vi "libssh2_knownhost_readfile.vi"(8 "error in (no error)":errorcluster, 9 "type (OpenSSH)":T1, 10 "filename":path, 11 "host key database":T2) -> (0 "error out":errorcluster, 2 "hosts added":i32)   [LabVIEW 2017, in "libssh2.lvlib"]
doc: "Read host keys from a file and add them to a host key database."
uses:
  libssh2.lvlib
  Host Key Database Refnum.ctl
  Host Key File Type.ctl
  Not A Host Key Database.vi
  <vilib>/Utility/error.llb/Error Cluster From Error Code.vi
  Global Settings.vi
  Read Host Key Database Refnum.vi
  <vilib>/Utility/semaphor.llb/Acquire Semaphore.vi
  <vilib>/Utility/semaphor.llb/Release Semaphore.vi
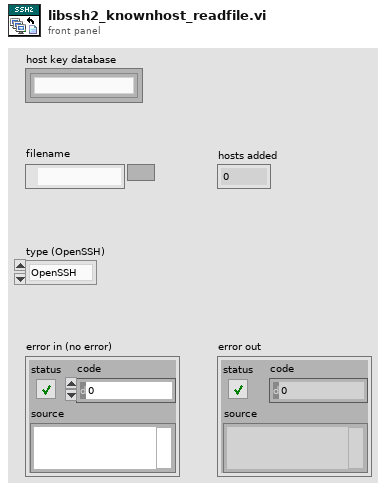
[diagram p1: front panel]
types:
  T1 = typedef "libssh2.lvlib/Host Key File Type.ctl" = enum16{"OpenSSH"}
  T2 = typedef "libssh2.lvlib/Host Key Database Refnum.ctl" = refnum<k1>
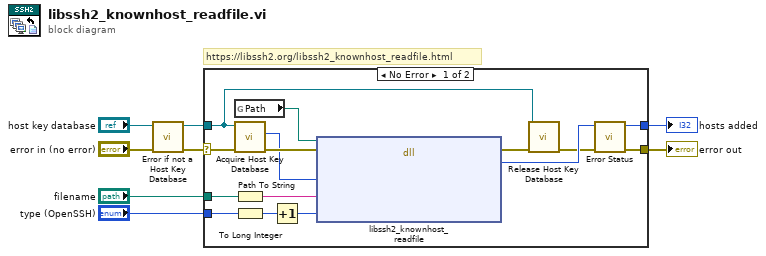
[diagram p0: block diagram]
diagram:
  # "https://libssh2.org/libssh2_knownhost_readfile.html"
  n1 = call "Error if not a Host Key Database.vi"("error in (no error)"="error in (no error)", "host key database"="host key database") -> ("error out"=w3:errorcluster, "host key database out"=w1:T2)  [unwired: 8 in]
  n2 = case shown="No Error" w3 {
    selector: w3 -> [w21 w24]
    tunnel: [w19 _] -> w8
    tunnel: [w20 w24] -> w7
    tunnel: "filename" -> [w23 _]
    tunnel: "type (OpenSSH)" -> [w22 _]
    tunnel: w1 -> [w9 _]
    frame No Error {
      n3 = global read "Global Settings.vi" "Path"() -> (w15:path)
      n4 = call "Acquire Host Key Database.vi"("error in (no error)"=w21, "host key database"=w9) -> ("error out"=w17:errorcluster, "LIBSSH2_KNOWNHOSTS*"=w16:u64)  [unwired: 8 in]
      n5 = Path To String(path=w23) -> (string=w13:string)
      n6 = To Long Integer(number=w22) -> (32bit integer=w11:i32)
      n7 = Increment(x=w11) -> (x+1=w12:i32)
      n8 = dll-call lib="?" fn="libssh2_knownhost_readfile"(path in=w15, error in=w17, "hosts"=w16, "filename"=w13, "type"=w12) -> (error out=w18:errorcluster, "return value"=w14:i32)  [unwired: 4 in, 1 out]
      n9 = call "Release Host Key Database.vi"("error in (no error)"=w18, "host key database"=w9) -> ("error out"=w10:errorcluster)  [unwired: 9 in]
      n10 = call "Error Status.vi"("error in (no error)"=w10, "return value"=w14) -> ("error out"=w20:errorcluster, "return value out"=w19:i32)  [unwired: 8 in]
    }
    frame Error {
    }
  }
  "hosts added" <- w8
  "error out" <- w7
